vi "anyfix.vi"() -> ()   [LabVIEW 2020]
panel:
  out "?":dbl
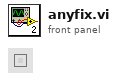
[diagram p1: front panel]
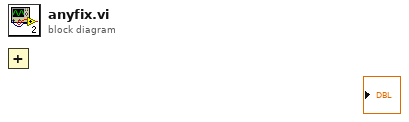
[diagram p0: block diagram]
diagram:
  n1 = Add() -> ()  [unwired: 2 in, 1 out]
